vi "ZAdania 2.vi"() -> ()   [LabVIEW 2025]
panel:
  out "Waveform Graph 2":cluster{"y":dbl, dbl, dbl[][]}(graph)
  out "Waveform Graph":dbl[](graph)
  out "Waveform Chart":dbl(graph)
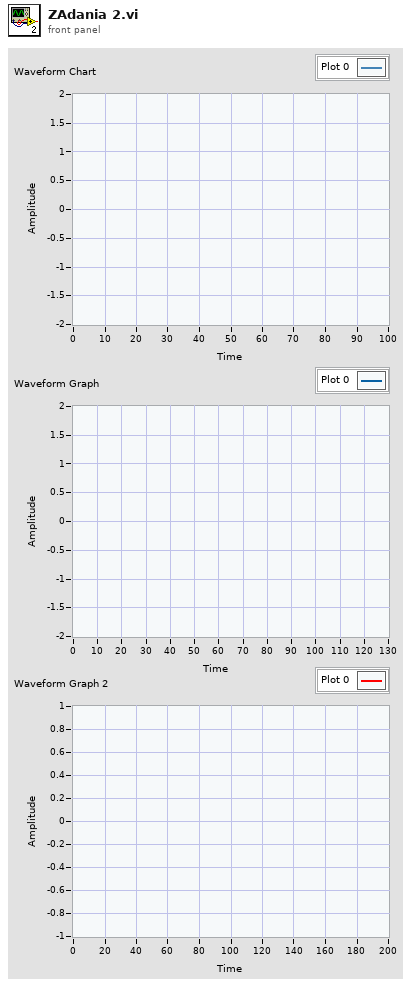
[diagram p1: front panel]
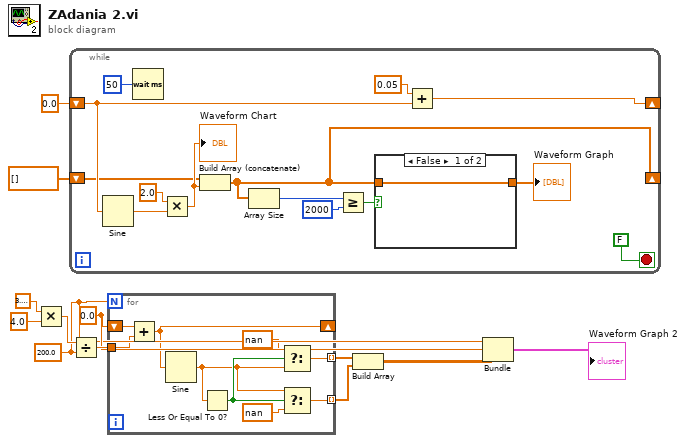
[diagram p0: block diagram]
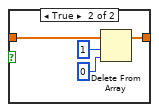
[diagram p2: hidden frame]
diagram:
  w2 = 200.0 ("y")
  w3 = 0.0
  n1 = Multiply(x=3.141592653589793, y=4.0) -> (x*y=w8:dbl)
  n2 = while {
    shift-right: [w23] -> _
    shift-left: 0.0 -> [w25]
    shift-right: [w13] -> _
    shift-left: dbl[] [] ("Array") -> [w18]
    stop <- FALSE stop-if-true
    n3 = Sine(x=w25) -> (sin(x)=w21:dbl)
    n4 = Wait (ms)(milliseconds to wait=u32 50) -> ()  [unwired: 1 out]
    n5 = Multiply(x=2.0, y=w21) -> (x*y=w19:dbl)
    "Waveform Chart" <- w19
    n6 = Build Array (concatenate)(w18, w19) -> (w13:dbl[])
    n7 = Array Size(array=w13) -> (size(s)=w17:i32)
    n8 = Greater Or Equal?(x=w17, y=2000) -> (x >= y?=w15:bool)
    n9 = case shown="False" w15 {
      tunnel: w13 -> [w27 w29]
      tunnel: [w27 w28] -> w14
      frame False {
      }
      frame True {
        n10 = Delete From Array(array=w29, length=1, index=0) -> (array with subset deleted=w28:dbl[])  [unwired: 1 out]
      }
    }
    "Waveform Graph" <- w14
    n11 = Add(x=0.05, y=w25) -> (x+y=w23:dbl)
  }
  n12 = Divide(x=w8, y=w2) -> (x/y=w7:dbl)
  n13 = for {
    N: w2 -> [_]
    shift-right: [w38] -> _
    shift-left: w3 -> [w40]
    tunnel: w7 -> [w39]
    tunnel: [w36] -> w5 mode=indexing
    tunnel: [w32] -> w6 mode=indexing
    n14 = Add(x=w40, y=w39) -> (x+y=w38:dbl)
    n15 = Sine(x=w38) -> (sin(x)=w34:dbl)
    n16 = Less Or Equal To 0?(x=w34) -> (x <= 0?=w35:bool)
    n17 = Select(t=nan, s=w35, f=w34) -> (s? t:f=w36:dbl)
    n18 = Select(t=w34, s=w35, f=nan) -> (s? t:f=w32:dbl)
  }
  n19 = Build Array(w5, w6) -> (w4:dbl[][])
  n20 = Bundle("y"=w2, w3, w4) -> (→"Waveform Graph 2":cluster{"y":dbl, dbl, dbl[][]})  [unwired: 1 in]
